vi "SubVI Drehung.vi"() -> ()   [LabVIEW 2015]
uses:
  <vilib>/NXT/Block Support/NXT_OutputPort.ctl
  <vilib>/NXT/LegoClasses/BrickReference/BrickReference.lvclass
  <vilib>/NXT/Subs/LVHSConnector.ctl
  <vilib>/NXT/NXTIO Xnodes/NXTIOXNode/NXTIO.xnode
  <vilib>/NXT/NXTIO Xnodes/AddressXNode/NXTIOAddress.xnode
  <vilib>/NXT/Block Support/NXT_InputPort.ctl
  <vilib>/NXT/Dual Mode Library/Sensors/EV3_Gyro_Angle.vi
  <vilib>/NXT/NXTIO Xnodes/NXTIONodeSubVIs/NXTStopMotors.vi
  <vilib>/NXT/NXTIO Xnodes/NXTIONodeSubVIs/LEGOMoveAllMotors.vi
  <vilib>/NXT/NXTIO Xnodes/NXTIONodeSubVIs/NXTMoveMotors.vi
panel:
  in  "Wunschwinkel (St.0)":dbl
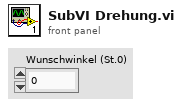
[diagram p1: front panel]
types:
  T1 = typedef "NXT_InputPort.ctl" = u32
  T2 = typedef "LVHSConnector.ctl" = refnum<class "BrickReference.lvclass">
  T3 = typedef "NXT_OutputPort.ctl" = u8
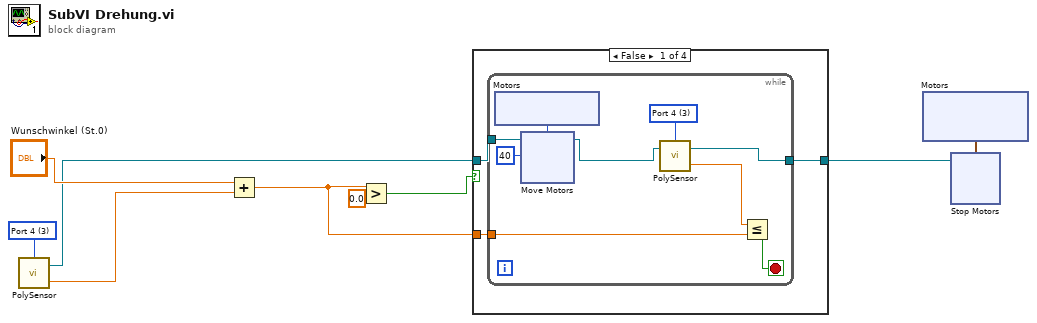
[diagram p0: block diagram]
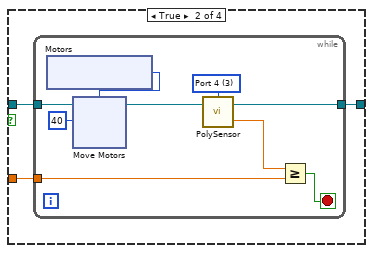
[diagram p2: hidden frame]
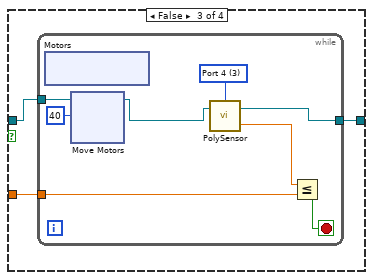
[diagram p3: hidden frame]
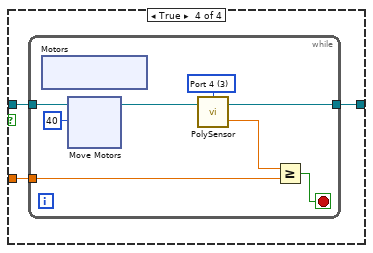
[diagram p4: hidden frame]
diagram:
  w6 = T1 3 items=["Port 1", "Port 2", "Port 3", "Port 4"] ("Port (Port 1)")
  n1 = call-poly <vilib>:"PolySensor.vi"("Port (Port 1)"=w6) -> ("Degrees"=w4:sgl, "NXT/EV3"=w1:T2)  [unwired: 2 in]
  n2 = Add(x="Wunschwinkel (St.0)", y=w4) -> (x+y=w3:dbl)
  n3 = Greater?(x=w3, y=0.0) -> (0:w2:bool)
  n4 = case shown="False" w2 {
    tunnel: [w12 w32 w50 w69] -> w8
    tunnel: w3 -> [w11 w31 w52 w70]
    tunnel: w1 -> [w10 w30 w51 w71]
    frame False {
      n5 = while {
        tunnel: [w20] -> w12
        tunnel: w11 -> [w18]
        tunnel: w10 -> [w14]
        stop <- w15 stop-if-true
        w17 = T1 3 items=["Port 1", "Port 2", "Port 3", "Port 4"] ("Port (Port 1)")
        n6 = xnode "Motors"() -> ("Motor"=w13:T3)
        n7 = xnode "Move Motors"("Power/Speed 1"=i8 40, "Motors"=w13, "NXT/EV3"=w14) -> ("NXT/EV3"=w21:T2)
        n8 = call-poly <vilib>:"PolySensor.vi"("NXT/EV3"=w21, "Port (Port 1)"=w17) -> ("Degrees"=w16:sgl, "NXT/EV3"=w20:T2)  [unwired: 1 in]
        n9 = Less Or Equal?(x=w16, y=w18) -> (x <= y?=w15:bool)
      }
    }
    frame True {
      n10 = while {
        tunnel: [w40] -> w32
        tunnel: w31 -> [w38]
        tunnel: w30 -> [w34]
        stop <- w35 stop-if-true
        w37 = T1 3 items=["Port 1", "Port 2", "Port 3", "Port 4"] ("Port (Port 1)")
        n11 = xnode "Motors"() -> ("Motor"=w33:T3)
        n12 = xnode "Move Motors"("Power/Speed 1"=i8 40, "Motors"=w33, "NXT/EV3"=w34) -> ("NXT/EV3"=w41:T2)
        n13 = call-poly <vilib>:"PolySensor.vi"("NXT/EV3"=w41, "Port (Port 1)"=w37) -> ("Degrees"=w36:sgl, "NXT/EV3"=w40:T2)  [unwired: 1 in]
        n14 = Greater Or Equal?(x=w36, y=w38) -> (x >= y?=w35:bool)
      }
    }
    frame False {
      n15 = while {
        tunnel: [w59] -> w50
        tunnel: w52 -> [w57]
        tunnel: w51 -> [w53]
        stop <- w54 stop-if-true
        w56 = T1 3 items=["Port 1", "Port 2", "Port 3", "Port 4"] ("Port (Port 1)")
        n16 = xnode "Motors"() -> ()  [unwired: 1 out]
        n17 = xnode "Move Motors"("Power/Speed 1"=i8 40, "NXT/EV3"=w53) -> ("NXT/EV3"=w60:T2)  [unwired: 1 in]
        n18 = call-poly <vilib>:"PolySensor.vi"("NXT/EV3"=w60, "Port (Port 1)"=w56) -> ("Degrees"=w55:sgl, "NXT/EV3"=w59:T2)  [unwired: 1 in]
        n19 = Less Or Equal?(x=w55, y=w57) -> (x <= y?=w54:bool)
      }
    }
    frame True {
      n20 = while {
        tunnel: [w78] -> w69
        tunnel: w70 -> [w76]
        tunnel: w71 -> [w72]
        stop <- w73 stop-if-true
        w75 = T1 3 items=["Port 1", "Port 2", "Port 3", "Port 4"] ("Port (Port 1)")
        n21 = xnode "Motors"() -> ()  [unwired: 1 out]
        n22 = xnode "Move Motors"("Power/Speed 1"=i8 40, "NXT/EV3"=w72) -> ("NXT/EV3"=w79:T2)  [unwired: 1 in]
        n23 = call-poly <vilib>:"PolySensor.vi"("NXT/EV3"=w79, "Port (Port 1)"=w75) -> ("Degrees"=w74:sgl, "NXT/EV3"=w78:T2)  [unwired: 1 in]
        n24 = Greater Or Equal?(x=w74, y=w76) -> (x >= y?=w73:bool)
      }
    }
  }
  n25 = xnode "Motors"() -> ("Motor"=w7:cluster{"Port":T3, "Port":T3})
  n26 = xnode "Stop Motors"("Motors"=w7, "NXT/EV3"=w8) -> ()  [unwired: 1 out]
